vi "Obtain Ready for Events Notifier.vi"(8 "error in (no error)":errorcluster) -> (0 "error out":errorcluster, 3 "notifier":refnum<notifier>)   [LabVIEW 2018, in "GLog.lvlib" / "Registry.lvlib"]
uses:
  Registry.lvlib
panel:
  # "Connector Pane"
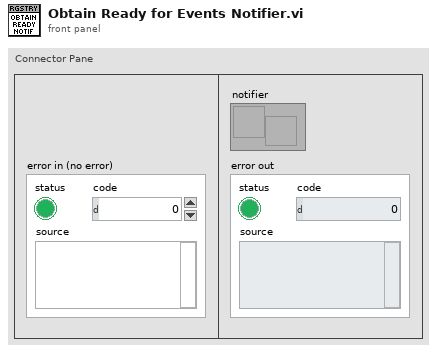
[diagram p1: front panel]
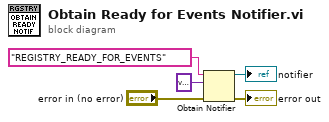
[diagram p0: block diagram]
diagram:
  n1 = Obtain Notifier(name (unnamed)="REGISTRY_READY_FOR_EVENTS", notification data type=variant, error in (no error)="error in (no error)") -> (notifier out=→"notifier":refnum<notifier>, error out=→"error out":errorcluster)  [unwired: 1 in, 1 out]
